vi "GpuMat Download_HostMem.vi"(8 "error in (no error)":errorcluster, 9 "Stream in":refnum<class "Stream.lvclass">, 10 "HostMem":refnum<class "HostMem.lvclass">, 11 "GpuMat in":refnum<class "GpuMat.lvclass">) -> (0 "error out":errorcluster, 1 "Stream out":refnum<class "Stream.lvclass">, 2 "HostMem out":refnum<class "HostMem.lvclass">, 3 "GpuMat out":refnum<class "GpuMat.lvclass">)   [LabVIEW 2020, in "OpenLvVision_OpenCv.lvlib" / "Cuda.lvlib" / "GpuMat.lvclass"]
doc: "Transfers data from the GPU device memory (GpuMat) back to a page-locked (pinned) host memory buffer (HostMem). Just like the upload function, using pinned memory accelerates the transfer. Providing a `Stream` reference allows this download to happen asynchronously."
uses:
  GpuMat.lvclass
  OpenLvVision_OpenCv.lvlib
  <vilib>/Utility/error.llb/Error Cluster From Error Code.vi
  <vilib>/ErrorRing/Error Ring.xnode
  _LvHelpers/EdvrObject/EdvrObject.lvclass
  Dlls/OlvOpenCvWrapper.dll
  Stream/Stream.lvclass
  C:/Users/lukas/Documents/OpenLvVision_OpenCv/SourceCode/LabView/OpenLvVision_OpenCv/_LvHelpers/EdvrObject/EdvrObject.lvclass
  C:/Users/lukas/Documents/OpenLvVision_OpenCv/SourceCode/LabView/OpenLvVision_OpenCv/Cuda/DataAccess/Stream/Stream.lvclass
  HostMem/HostMem.lvclass
  C:/Users/lukas/Documents/OpenLvVision_OpenCv/SourceCode/LabView/OpenLvVision_OpenCv/Cuda/DataAccess/HostMem/HostMem.lvclass
  C:/Users/lukas/Documents/OpenLvVision_OpenCv/SourceCode/LabView/OpenLvVision_OpenCv/Cuda/DataAccess/GpuMat/GpuMat.lvclass
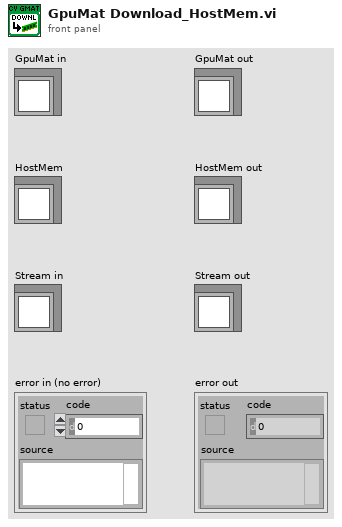
[diagram p1: front panel]
types:
  T1 = typedef "OpenLvVision_OpenCv.lvlib/EdvrObject.lvclass/Edvr.ctl" = refnum<data-value>
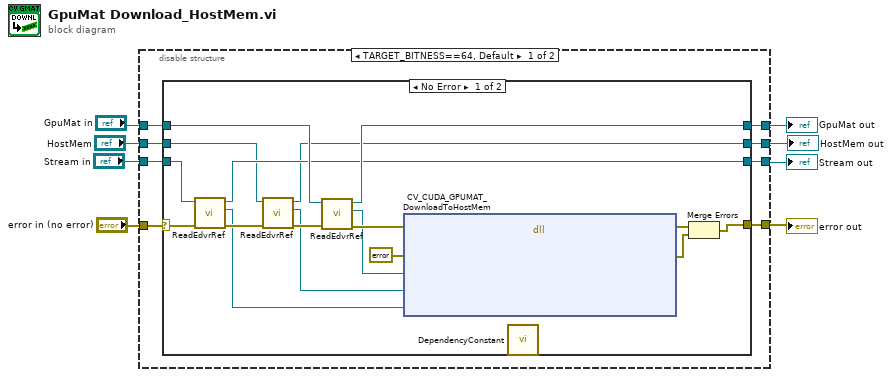
[diagram p0: block diagram]
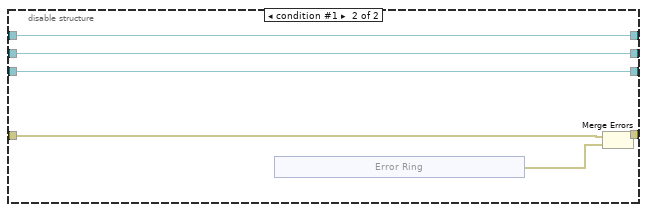
[diagram p3: hidden frame]
diagram:
  n1 = disable-structure shown="TARGET_BITNESS==64, Default" {
    disable-tunnel: "error in (no error)" -> [w16 w42]
    disable-tunnel: [w15 w43] -> w8
    disable-tunnel: "GpuMat in" -> [w14 w39]
    disable-tunnel: [w13 w39] -> w5
    disable-tunnel: "HostMem" -> [w12 w38]
    disable-tunnel: "Stream in" -> [w11 w40]
    disable-tunnel: [w10 w40] -> w2
    disable-tunnel: [w9 w38] -> w1
    frame condition #0 (active) {
      n2 = case shown="No Error" w16 {
        selector: w16 -> [w25 w37]
        tunnel: [w30 w37] -> w15
        tunnel: w14 -> [w28 w35]
        tunnel: [w26 w35] -> w13
        tunnel: w12 -> [w17 w34]
        tunnel: w11 -> [w22 w36]
        tunnel: [w19 w36] -> w10
        tunnel: [w18 w34] -> w9
        frame No Error {
          n3 = call "ReadEdvrRef.vi"("error in (no error)"=w25, "EdvrObject in"=w22) -> ("error out"=w24:errorcluster, "Edvr"=w20:T1, "EdvrObject out"=w19:refnum<class "Stream.lvclass">)  [unwired: 7 in]
          n4 = call "ReadEdvrRef.vi"("error in (no error)"=w24, "EdvrObject in"=w17) -> ("error out"=w23:errorcluster, "Edvr"=w21:T1, "EdvrObject out"=w18:refnum<class "HostMem.lvclass">)  [unwired: 7 in]
          n5 = call "ReadEdvrRef.vi"("error in (no error)"=w23, "EdvrObject in"=w28) -> ("error out"=w29:errorcluster, "Edvr"=w27:T1, "EdvrObject out"=w26:refnum<class "GpuMat.lvclass">)  [unwired: 7 in]
          n6 = dll-call lib="C:/Users/lukas/Documents/OpenLvVision_OpenCv/SourceCode/LabView/OpenLvVision_OpenCv/Dlls/OlvOpenCvWrapper.dll" fn="CV_CUDA_GPUMAT_DownloadToHostMem"(error in=w29, "Error"=errorcluster {"status"=FALSE, "code"=0, "source"=""} ("error out"), "edvrRef"=w27, "hostMemRef"=w21, "streamRef"=w20) -> (error out=w33:errorcluster, "Error"=w32:errorcluster)  [unwired: 6 in, 1 out]
          n7 = call "DependencyConstant.vi"() -> ()  [unwired: 12 in]
          n8 = Merge Errors(w33, w32) -> (w30:errorcluster)
        }
        frame Error {
        }
      }
    }
    frame condition #1 {
      n9 = xnode "Error Ring"() -> ("error out"=w41:errorcluster)
      n10 = Merge Errors(w42, w41) -> (w43:errorcluster)
    }
  }
  "error out" <- w8
  "GpuMat out" <- w5
  "Stream out" <- w2
  "HostMem out" <- w1
